vi "tdms_index_trans.vi"(11 "B_TDMS_Path_Temp":path) -> (3 "path":path)   [LabVIEW 2018]
panel:
  out "output array":string[](array[string])
  out "before substring":string
  out "element":string
  out "array of strings":string[](array[string])
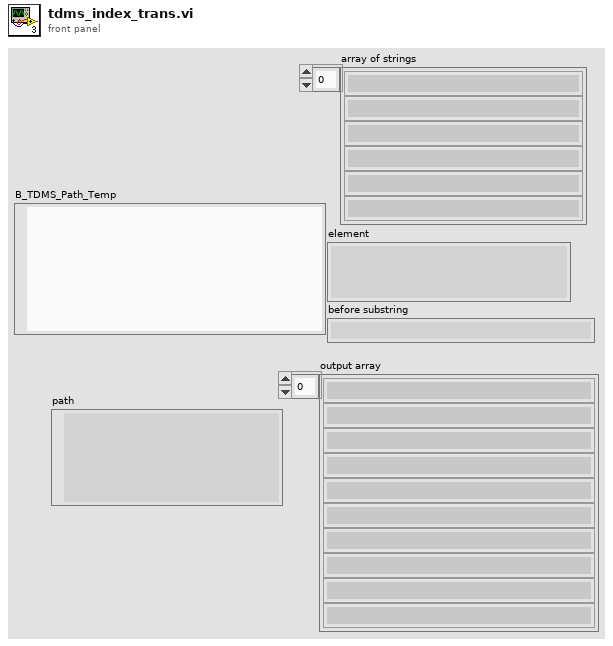
[diagram p1: front panel]
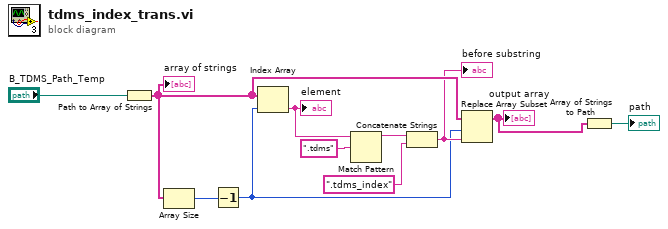
[diagram p0: block diagram]
diagram:
  n1 = Path to Array of Strings(0:"B_TDMS_Path_Temp") -> (2:w5:string[])  [unwired: 1 out]
  "array of strings" <- w5
  n2 = Array Size(array=w5) -> (size(s)=w10:i32)
  n3 = Decrement(x=w10) -> (x-1=w3:i32)
  n4 = Index Array(array=w5, index=w3) -> (element=w9:string)
  "element" <- w9
  n5 = Match Pattern(string=w9, regular expression=".tdms") -> (before substring=w7:string)  [unwired: 1 in, 3 out]
  n6 = Concatenate Strings(w7, ".tdms_index" ("string")) -> (w4:string)
  "before substring" <- w4
  n7 = Replace Array Subset(array=w5, new element=w4, index=w3) -> (w2:string[])
  "output array" <- w2
  n8 = Array of Strings to Path(0:w2) -> (2:→"path":path)  [unwired: 1 in]
